vi "Set Build Specification Version.vi"(6 "Build Specification Version":T1, 8 "error in":errorcluster, 9 "Build Specification":string, 10 "Project File":path, 11 "IProject Manager in":refnum<class "Mock IProject Manager.lvclass">) -> (0 "error out":errorcluster, 3 "IProject Manager out":refnum<class "Mock IProject Manager.lvclass">)   [LabVIEW 2026, in "Mock IProject Manager.lvclass"]
doc: "Set version of PPL build specification."
uses:
  Mock IProject Manager.lvclass
  C:/Program Files/National Instruments/LabVIEW 2026/vi.lib/Astemes/LMock/Mock.lvclass
  <vilib>/AppBuilder/AB_API_Simple/Build Specification Version.ctl
  <vilib>/Astemes/LMock/Mock.lvclass
  <vilib>/AppBuilder/AB_API_Simple/NI_App_Builder_API.lvlib
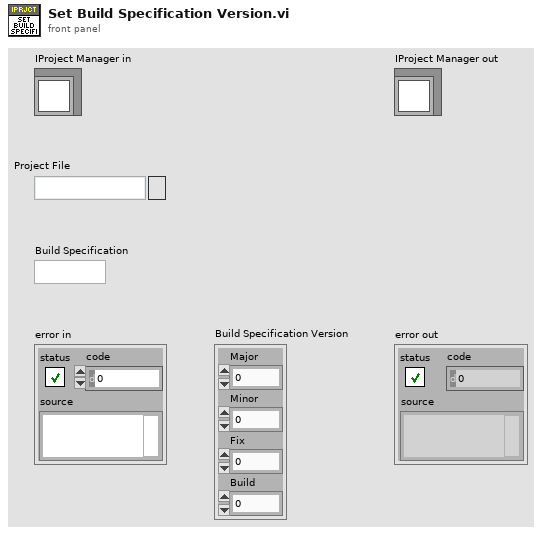
[diagram p1: front panel]
types:
  T1 = typedef "NI_App_Builder_API.lvlib/Build Specification Version.ctl" = cluster{"Major":u16, "Minor":u16, "Fix":u16, "Build":u16}
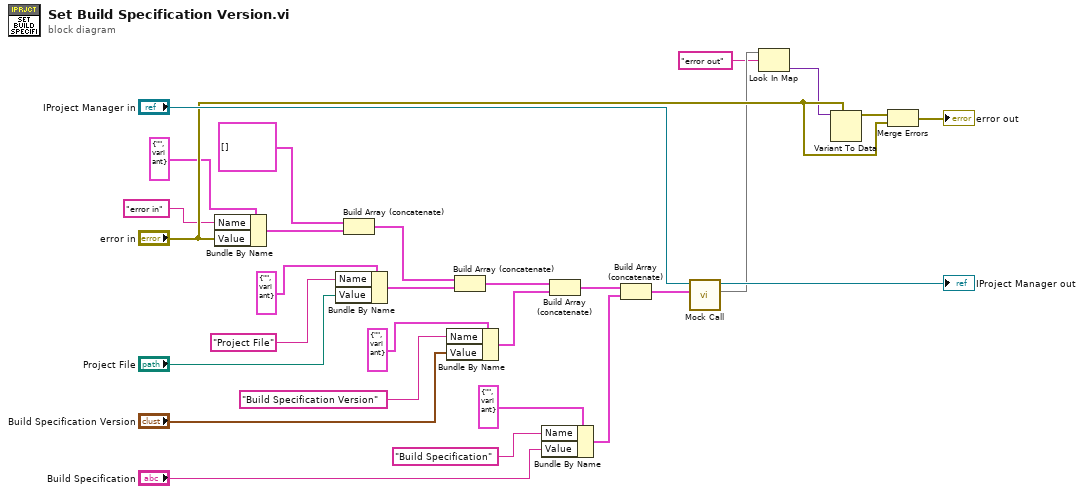
[diagram p0: block diagram]
diagram:
  n1 = Bundle By Name(cluster=cluster{"Name":string, "Value":variant} {"Name"="", "Value"=variant} ("element"), "Name"="error in", "Value"="error in") -> (w7:cluster{"Name":string, "Value":variant})
  n2 = Bundle By Name(cluster=cluster{"Name":string, "Value":variant} {"Name"="", "Value"=variant} ("element"), "Name"="Project File", "Value"="Project File") -> (w5:cluster{"Name":string, "Value":variant})
  n3 = Build Array (concatenate)(cluster{"Name":string, "Value":variant}[] [] ("Control Values"), w7) -> (w16:cluster{"Name":string, "Value":variant}[])
  n4 = Bundle By Name(cluster=cluster{"Name":string, "Value":variant} {"Name"="", "Value"=variant} ("element"), "Name"="Build Specification Version", "Value"="Build Specification Version") -> (w3:cluster{"Name":string, "Value":variant})
  n5 = Build Array (concatenate)(w16, w5) -> (w19:cluster{"Name":string, "Value":variant}[])
  n6 = Bundle By Name(cluster=cluster{"Name":string, "Value":variant} {"Name"="", "Value"=variant} ("element"), "Name"="Build Specification", "Value"="Build Specification") -> (w1:cluster{"Name":string, "Value":variant})
  n7 = Build Array (concatenate)(w19, w3) -> (w22:cluster{"Name":string, "Value":variant}[])
  n8 = Build Array (concatenate)(w22, w1) -> (w25:cluster{"Name":string, "Value":variant}[])
  n9 = call <vilib>:"Mock Call.vi"("Control Values"=w25, "Mock In"="IProject Manager in") -> ("Return Values"=w14:map{string, variant}, "Mock Out"=→"IProject Manager out":refnum<class "Mock IProject Manager.lvclass">)  [unwired: 8 in]
  n10 = Look In Map(map=w14, key="error out") -> (value=w12:variant)  [unwired: 1 in, 1 out]
  n11 = Variant To Data(type="error in", Variant=w12) -> (data=w11:errorcluster)  [unwired: 1 in, 1 out]
  n12 = Merge Errors(w11, "error in") -> (→"error out":errorcluster)
